vi "Read TOML File (LV).vi"(7 "Default Value":variant, 8 "error in (no error)":errorcluster, 11 "file path (use dialog)":path) -> (0 "error out":errorcluster, 3 "Value":variant)   [LabVIEW 2015, in "TOML.lvlib"]
uses:
  TOML.lvlib
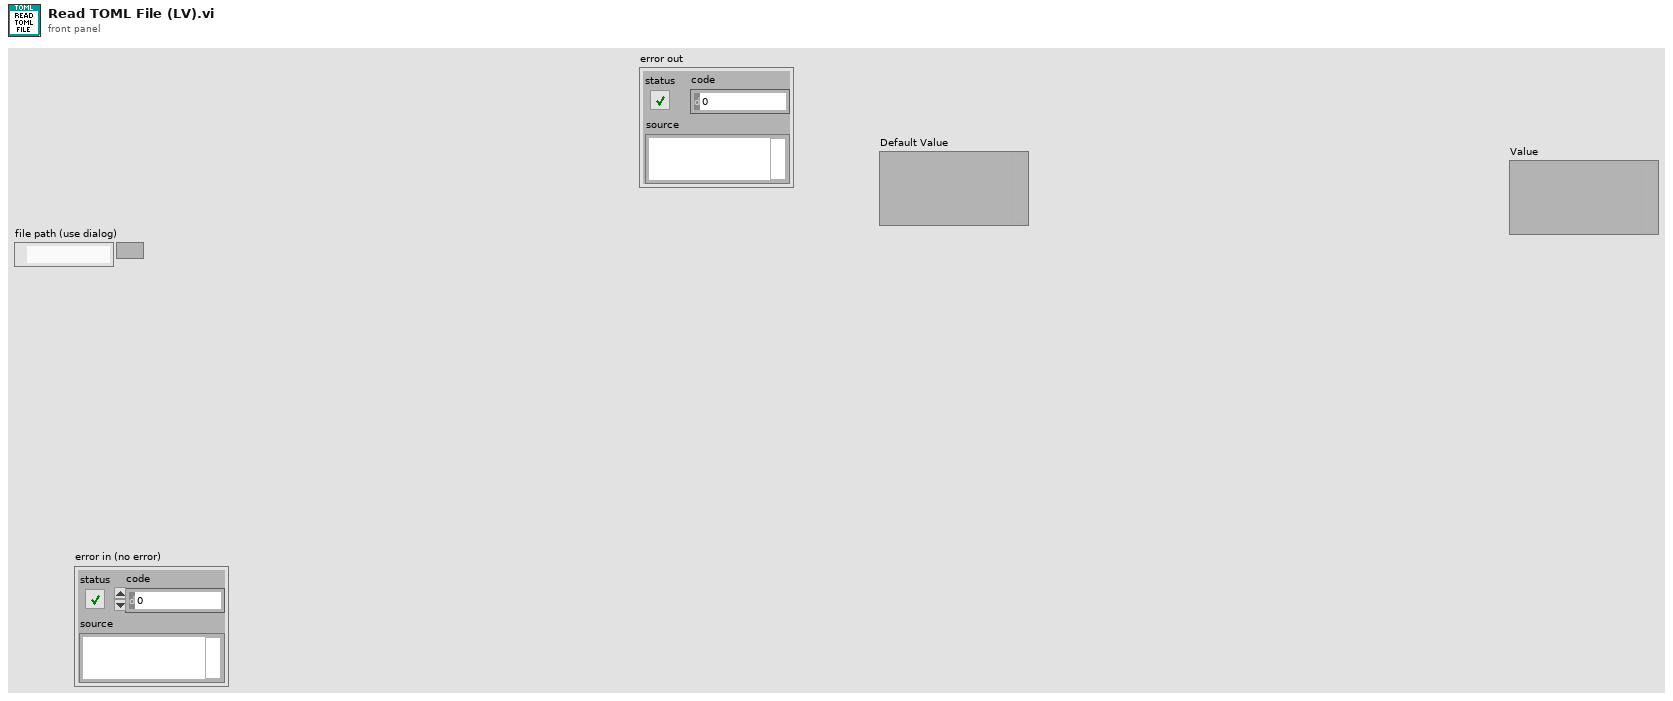
[diagram p1: front panel]
types:
  T1 = enum16{"open", "replace", "create", "open or create", "replace or create", "replace or create with confirmation"}
  T2 = typedef "TOML.lvlib/TOML Value.ctl" = cluster{"\\type":enum16{"Table", "Array", "String", "Integer", "Float", "Boolean", "Offset Date-Time", "Local Date-Time", "Local Date", "Local Time"}, "ÿýÿýÿýÿýÿýÿþÿýÿýÿý%LV-TOML.lvlib:TOML Key-Value Pair.ctlÿýÿýÿýÿýÿýÿþÿýÿýÿýLV-TOML.lvlib:TOML Value.ctl$":variant}
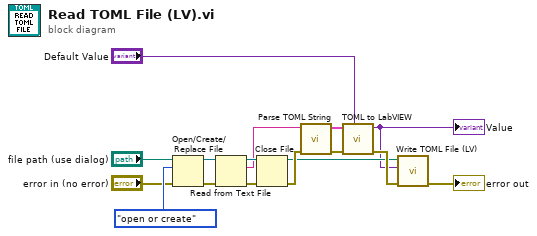
[diagram p0: block diagram]
diagram:
  n1 = Open/Create/Replace File(file path (use dialog)="file path (use dialog)", error in="error in (no error)", operation (0:open)=T1."open or create") -> (refnum out=w13:refnum<file>, error out=w14:errorcluster)  [unwired: 3 in, 1 out]
  n2 = Read from Text File(file (use dialog)=w13, error in=w14) -> (refnum out=w11:refnum<file>, text=w9:string, error out=w12:errorcluster)  [unwired: 2 in, 1 out]
  n3 = Close File(refnum=w11, error in=w12) -> (path=w3:path, error out=w8:errorcluster)
  n4 = call "Parse TOML String.vi"("error in (no error)"=w8, "String"=w9) -> ("error out"=w6:errorcluster, "Value"=w1:T2)  [unwired: 8 in]
  n5 = call "TOML to LabVIEW.vi"("Default Value"="Default Value", "error in (no error)"=w6, "TOML Value"=w1) -> ("error out"=w5:errorcluster, "LV Value"=w2:variant)  [unwired: 7 in]
  "Value" <- w2
  n6 = call "Write TOML File (LV).vi"("error in (no error)"=w5, "Value"=w2, "file path (use dialog)"=w3) -> ("error out"=→"error out":errorcluster)  [unwired: 8 in]
